vi "Set Topic Attribute.vi"(8 "error in (no error)":errorcluster, 10 "Topic Attribute":T1, 11 "Topic":refnum<class "Topic.lvclass">) -> (0 "error out":errorcluster, 3 "Topic out":refnum<class "Topic.lvclass">)   [LabVIEW 2015, in "NI_AWS_SNS.lvlib" / "Topic.lvclass"]
doc: "Allows a topic owner to set an attribute of the topic to a new value."
uses:
  Topic.lvclass
  Mutable Topic Attribute Value Pair.ctl
  Mutable Topic Attribute.ctl
  Core/HTTP Request/Request Options.ctl
  Core/HTTP Request/Name Value Pair.ctl
  Core/HTTP Request/Region handling.ctl
  Core/HTTP Request/URL formatting.ctl
  Core/ARN/ARN.lvclass/ARN.ctl
  Core/ARN/Read ARN.vi
  Core/HTTP Request/HTTP Request.lvclass
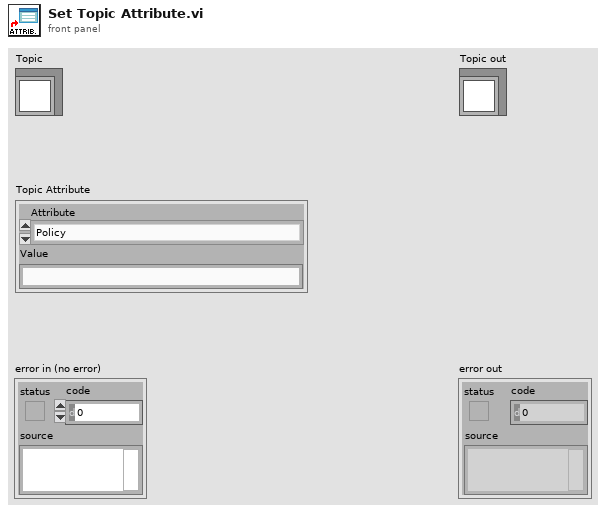
[diagram p1: front panel]
types:
  T1 = typedef "NI_AWS_SNS.lvlib/Topic.lvclass/Mutable Topic Attribute Value Pair.ctl" = cluster{"Attribute":T2, "Value":string}
  T2 = typedef "NI_AWS_SNS.lvlib/Topic.lvclass/Mutable Topic Attribute.ctl" = enum16{"Policy", "DisplayName", "DeliveryPolicy"}
  T3 = typedef "NI_AWS_Core.lvlib/HTTP Request.lvclass/Name Value Pair.ctl" = cluster{"name":string, "value":string}
  T4 = typedef "NI_AWS_Core.lvlib/HTTP Request.lvclass/Request Options.ctl" = cluster{"request headers":T3[], "request parameters":T3[], "request body":string, "region handling":T5, "URL formatting":T6}
  T5 = typedef "NI_AWS_Core.lvlib/HTTP Request.lvclass/Region handling.ctl" = enum16{"use region everywhere", "use region (authentication only)", "use region (URL only)", "ignore region everwhere"}
  T6 = typedef "NI_AWS_Core.lvlib/HTTP Request.lvclass/URL formatting.ctl" = enum16{"region-", "region."}
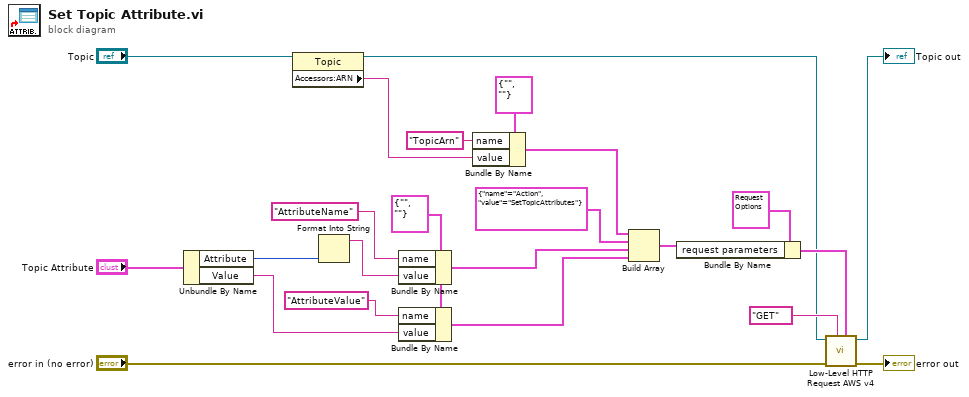
[diagram p0: block diagram]
diagram:
  w7 = T3 {"name"="", "value"=""} ("element")
  n1 = Unbundle By Name("Topic Attribute") -> ("Attribute"=w10:T2, "Value"=w5:string)
  n2 = property class="Topic"(reference="Topic") -> (reference out=w1:refnum<class "Topic.lvclass">, "Accessors:ARN"=w12:string)  [unwired: 1 in, 1 out]
  n3 = Format Into String(w10) -> (resulting string=w8:string)  [unwired: 3 in, 1 out]
  n4 = Bundle By Name(cluster=w7, "name"="AttributeName", "value"=w8) -> (w16:T3)
  n5 = Bundle By Name(cluster=w7, "name"="AttributeValue", "value"=w5) -> (w15:T3)
  n6 = Bundle By Name(cluster=T3 {"name"="", "value"=""} ("element"), "name"="TopicArn", "value"=w12) -> (w11:T3)
  n7 = Build Array(w11, T3 {"name"="Action", "value"="SetTopicAttributes"} ("Cluster"), w16, w15) -> (w17:T3[])
  n8 = Bundle By Name(cluster=T4 {"request headers"=[], "request parameters"=[{"name"="Action", "value"="ListQueues"}], "request body"="", "region handling"=enum."use region everywhere", "URL formatting"=enum."region."} ("Request Options"), "request parameters"=w17) -> (w3:T4)
  n9 = call "Low-Level HTTP Request AWS v4.vi"("Request Options"=w3, "HTTP-Verb"="GET", "error in (no error)"="error in (no error)", "AWS Core in"=w1) -> ("error out"=→"error out":errorcluster, "AWS Core out"=→"Topic out":refnum<class "Topic.lvclass">)  [unwired: 4 in, 2 out]
